vi "grabar.vi"(5 "Save Data":bool, 6 "output cluster":T1, 7 "Bool Refnum in":refnum<vi>, 8 "error in (no error)":errorcluster, 9 "Record":bool, 10 "queue in":refnum<queue>, 11 "Boolean in":refnum<vi>) -> (0 "error out":errorcluster, 3 "Queue out":refnum<queue>)   [LabVIEW 2013]
uses:
  data.ctl
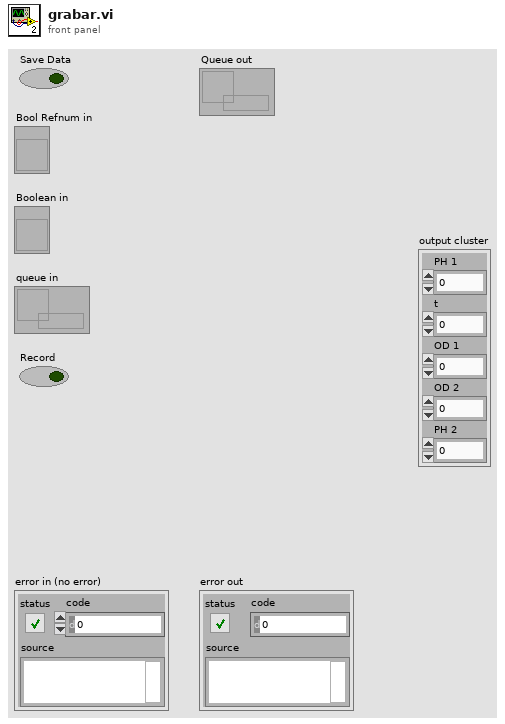
[diagram p1: front panel]
types:
  T1 = typedef "data.ctl" = cluster{"PH 1":dbl, "t":dbl, "OD 1":dbl, "OD 2":dbl, "PH 2":dbl}
  T2 = enum8{"Enabled", "Disabled", "Disabled and Grayed Out"}
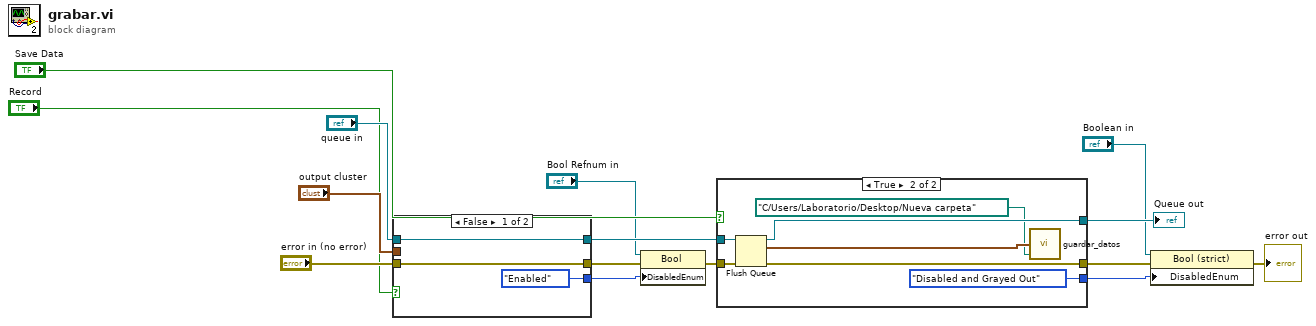
[diagram p0: block diagram]
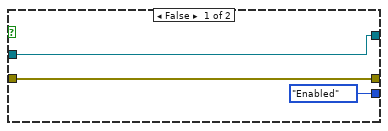
[diagram p2: hidden frame]
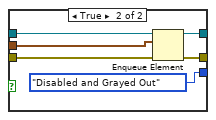
[diagram p3: hidden frame]
diagram:
  n1 = case shown="False" "Record" {
    tunnel: "queue in" -> [w18 w24]
    tunnel: [w18 w23] -> w5
    tunnel: "error in (no error)" -> [w17 w22]
    tunnel: [w17 w21] -> w12
    tunnel: "output cluster" -> [_ w20]
    tunnel: [T2."Enabled" ("Disabled") T2."Disabled and Grayed Out" ("Disabled")] -> w11
    frame False {
    }
    frame True {
      n2 = Enqueue Element(queue=w24, element=w20, error in (no error)=w22) -> (queue out=w23:refnum<queue>, error out=w21:errorcluster)  [unwired: 1 in, 1 out]
    }
  }
  n3 = property on="Property Node" class="Bool"(reference="Bool Refnum in", error in=w12, "DisabledEnum"=w11) -> (error out=w13:errorcluster)  [unwired: 1 out]
  n4 = case shown="True" "Save Data" {
    tunnel: w5 -> [w27 w34]
    tunnel: [w27 w33] -> w6
    tunnel: w13 -> [w26 w32]
    tunnel: [w26 w31] -> w14
    tunnel: [T2."Enabled" ("Disabled") T2."Disabled and Grayed Out" ("Disabled")] -> w10
    frame False {
    }
    frame True {
      n5 = Flush Queue(queue=w34, error in (no error)=w32) -> (queue out=w33:refnum<queue>, remaining elements=w30:T1[], error out=w31:errorcluster)
      n6 = call "guardar_datos.vi"("Path"=path "C:/Users/Laboratorio/Desktop/Nueva carpeta", "remaining elements"=w30) -> ()  [unwired: 2 in]
    }
  }
  "Queue out" <- w6
  n7 = property on="Property Node" class="Bool (strict)"(reference="Boolean in", error in=w14, "DisabledEnum"=w10) -> (error out=→"error out":errorcluster)  [unwired: 1 out]
